vi "GetClientComplexityv2.vi"() -> ()   [LabVIEW 2017]
uses:
  <vilib>/httpClient/LabVIEWHTTPClient.lvlib
  <vilib>/httpClient/POSTBuffer.vi
panel:
  out "error out":errorcluster
  out "test_property":T1
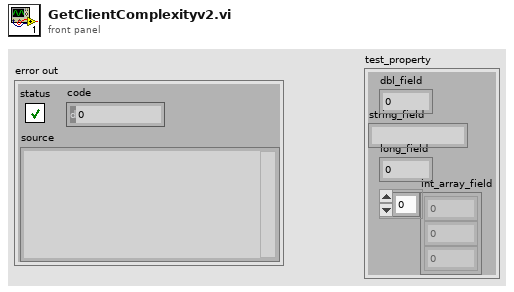
[diagram p1: front panel]
types:
  T1 = cluster{"dbl_field":dbl, "string_field":string, "long_field":i64, "int_array_field":i32[]}
  T2 = cluster{"req_action":string, "selector":string, "req_lang":string, "device":string, "type_descriptor":i16[]}
  T3 = typedef "LabVIEWHTTPClient.lvlib/ClientHandle.ctl" = refnum<k1>
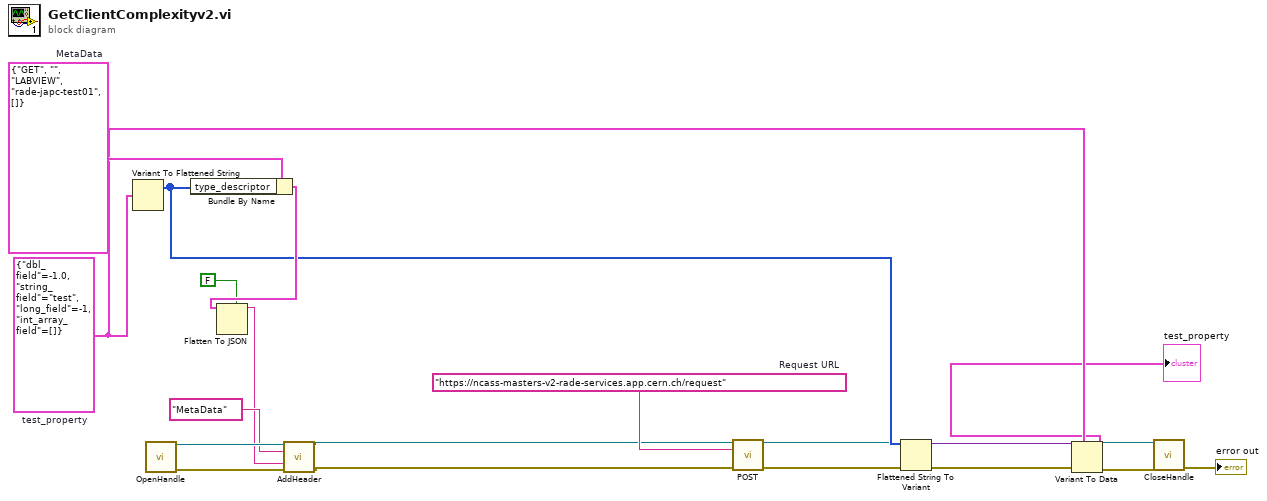
[diagram p0: block diagram]
diagram:
  w10 = "https://ncass-masters-v2-rade-services.app.cern.ch/request"  # Request URL
  w15 = T2 {"req_action"="GET", "selector"="", "req_lang"="LABVIEW", "device"="rade-japc-test01", "type_descriptor"=[]}  # MetaData
  w11 = T1 {"dbl_field"=-1.0, "string_field"="test", "long_field"=-1, "int_array_field"=[]}  # test_property
  n1 = Variant To Flattened String(Variant=w11) -> (1:w6:i16[])  [unwired: 1 out]
  n2 = call <vilib>:"OpenHandle.vi"() -> ("client handle out"=w18:T3, "error out"=w19:errorcluster)  [unwired: 14 in]
  n3 = Bundle By Name(cluster=w15, "type_descriptor"=w6) -> (w14:T2)
  n4 = Flatten To JSON(enable LabVIEW extensions? (T)=FALSE, anything=w14) -> (JSON string=w12:string)  [unwired: 1 in, 1 out]
  n5 = call <vilib>:"AddHeader.vi"("client handle"=w18, "header"="MetaData", "value"=w12, "error in (no error)"=w19) -> ("client handle out"=w2:T3, "error out"=w1:errorcluster)  [unwired: 10 in]
  n6 = call-poly <vilib>:"POST.vi"("client handle"=w2, "url"=w10, "error in (no error)"=w1) -> ("client handle out"=w5:T3, "error out"=w4:errorcluster)  [unwired: 9 in, 2 out]
  n7 = Flattened String To Variant(4:w4, 7:w6) -> (0:w7:errorcluster, 3:w8:variant)  [unwired: 1 in]
  n8 = Variant To Data(error in=w7, type=w11, Variant=w8) -> (data=→"test_property":T1, error out=w9:errorcluster)
  n9 = call <vilib>:"CloseHandle.vi"("client handle"=w5, "error in (no error)"=w9) -> ("error out"=→"error out":errorcluster)  [unwired: 13 in]
